vi "Remove Page.vi"(8 "error in (no error)":errorcluster, 10 "Page Name":string, 11 "Document in":refnum<class "Document.lvclass">) -> (0 "error out":errorcluster, 3 "Document out":refnum<class "Document.lvclass">)   [LabVIEW 2017, in "LabVIEW NPOI.lvlib" / "Document.lvclass"]
doc: "Removes page with the given <b>Page Name</b> from the <b>Document</b>."
uses:
  Document.lvclass
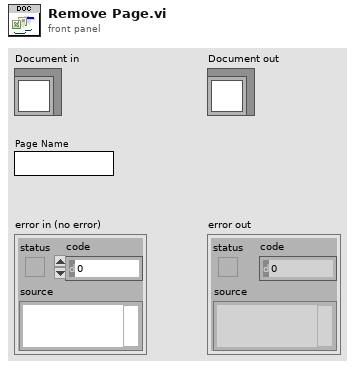
[diagram p1: front panel]
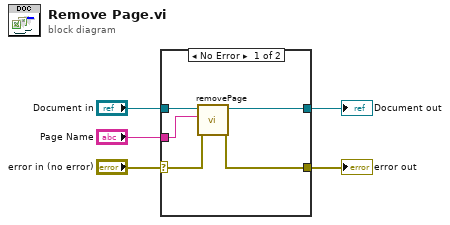
[diagram p0: block diagram]
diagram:
  n1 = case shown="No Error" "error in (no error)" {
    selector: "error in (no error)" -> [w7 w12]
    tunnel: [w6 w12] -> w4
    tunnel: [w9 w11] -> w2
    tunnel: "Document in" -> [w10 w11]
    tunnel: "Page Name" -> [w8 _]
    frame No Error {
      n2 = call-dynamic "removePage.vi"("error in (no error)"=w7, "Page Name"=w8, "Document in"=w10) -> ("error out"=w6:errorcluster, "Document out"=w9:refnum<class "Document.lvclass">)  [unwired: 7 in]
    }
    frame Error {
    }
  }
  "error out" <- w4
  "Document out" <- w2
